vi "subGenerateDGMLOtherFilesFolderString.vi"(7 "ILabVIEWItem in":refnum<class "ILabVIEWItem.lvclass">, 8 "Links in":T1, 9 "Nodes in":T1, 11 "CGrapherDGML in":refnum<class "CGrapherDGML.lvclass">) -> (0 "Links":T1, 1 "Nodes":T1, 2 "Path":string="Z:\\OtherFiles", 3 "CGrapherDGML":refnum<class "CGrapherDGML.lvclass">)   [LabVIEW 2020, in "DefaultExtensions.lvlib" / "CGrapherDGML.lvclass"]
uses:
  CGrapherDGML.lvclass
  LabVIEWObjectInterfaces/ILabVIEWItem/ILabVIEWItem.lvclass
  LabVIEWItem/CLabVIEWItem/ConnectionSet.ctl
  CGrapherDGML.lvclass/CGrapherDGML.ctl
  ecf4d353-cf80-4459-a486-8bebc84a9ab0.vi
  LabVIEWItem/CLabVIEWItem/CLabVIEWItem.lvclass
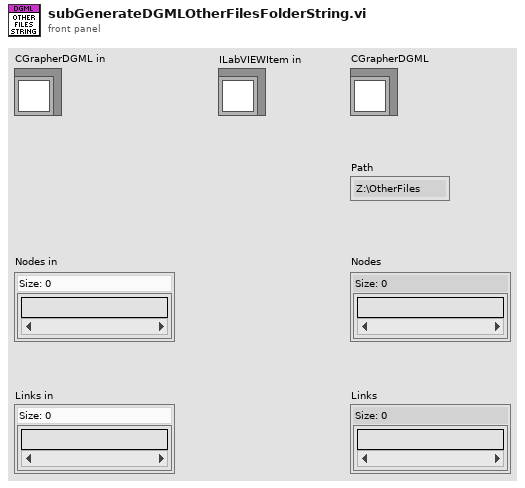
[diagram p1: front panel]
types:
  T1 = typedef "LabVIEWItem.lvlib/CLabVIEWItem.lvclass/ConnectionSet.ctl" = set{string}
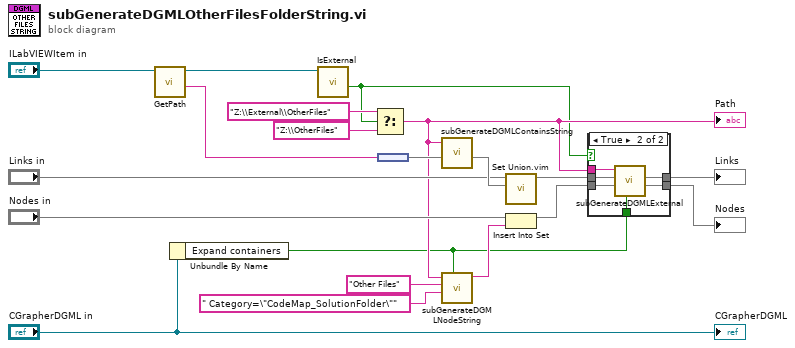
[diagram p0: block diagram]
diagram:
  n1 = call-dynamic "GetPath.vi"("ILabVIEWItem in"="ILabVIEWItem in") -> ("Path"=w20:string, "ILabVIEWItem out"=w14:refnum<class "ILabVIEWItem.lvclass">)  [unwired: 8 in, 1 out]
  n2 = Unbundle By Name("CGrapherDGML in") -> ("Expand containers"=w4:bool)
  n3 = call-dynamic "IsExternal.vi"("ILabVIEWItem in"=w14) -> ("Is external?"=w1:bool)  [unwired: 8 in, 2 out]
  n4 = Select(t="Z:\\External\\OtherFiles" ("format string"), s=w1, f="Z:\\OtherFiles" ("format string")) -> (s? t:f=w5:string)
  "Path" <- w5
  n5 = node(w20) -> (w19:set{string})
  n6 = call "subGenerateDGMLContainsString.vi"("Contained"=w19, "Source"=w5) -> ("Links"=w18:T1)  [unwired: 9 in]
  n7 = call "subGenerateDGMLNodeString.vi"("Expand?"=w4, "Code schema"=" Category=\"CodeMap_SolutionFolder\"" ("format string"), "Label"="Other Files" ("format string"), "Id"=w5) -> ("Node string"=w16:string)  [unwired: 7 in]
  n8 = call "Set Union.vim"("set 2"=w18, "set 1"="Links in") -> ("union"=w6:T1)  [unwired: 9 in]
  n9 = Insert Into Set(10:w16, 11:"Nodes in") -> (3:w7:T1)  [unwired: 1 out]
  n10 = case shown="True" w1 {
    tunnel: w7 -> [w21 w28]
    tunnel: w6 -> [w22 w27]
    tunnel: w5 -> [_ w26]
    tunnel: w4 -> [_ w25]
    tunnel: [w22 w24] -> w3
    tunnel: [w21 w23] -> w2
    frame False {
    }
    frame True {
      n11 = call "subGenerateDGMLExternal.vi"("Expand?"=w25, "Nodes in in"=w28, "union in"=w27, "format string"=w26) -> ("Nodes out"=w23:T1, "union out"=w24:T1)  [unwired: 6 in]
    }
  }
  "Links" <- w3
  "Nodes" <- w2
  "CGrapherDGML" <- "CGrapherDGML in"
